vi "_CSMObj-Add Internal Registry Rule.vi"(8 "Error In":errorcluster caption="error in (no error)", 10 "Rule":string, 11 "CSMQ In":T1={"info"={"Module Name"="", "Requested Name"="", "Group Name"="", "Mode"=enum."Stand Alone", "Allowed Messages"=[]}, "Refs"={"WatchDogQ"=refnum, "CSMDataDVR"=refnum, "Queue"={"HPriorityQ"=refnum, "LowPriorityQ"=refnum}, "GroupDataDVR"=refnum, "TagMap"=refnum, "ExitEvent"=refnum, "NewStateEvent"=refnum, "StatusEvent"=refnum, "InterruptEvent"=refnum}}) -> (0 "error out":errorcluster, 3 "CSMQ Out":T1={"info"={"Module Name"="", "Requested Name"="", "Group Name"="", "Mode"=enum."Stand Alone", "Allowed Messages"=[]}, "Refs"={"WatchDogQ"=refnum, "CSMDataDVR"=refnum, "Queue"={"HPriorityQ"=refnum, "LowPriorityQ"=refnum}, "GroupDataDVR"=refnum, "TagMap"=refnum, "ExitEvent"=refnum, "NewStateEvent"=refnum, "StatusEvent"=refnum, "InterruptEvent"=refnum}})   [LabVIEW 2017, in "Communicable State Machine.lvlib"]
uses:
  Communicable State Machine.lvlib
  _CSMObj.ctl
  _CSMObj-Info.ctl
  Typedef/_CSM_MODE.ctl
  _CSMObj-Refs.ctl
  _CSMObj-Data.ctl
  Priority Queue/Priority Queue.ctl
  Typedef/_Cross CSM State Data.ctl
  Typedef/_CSM_MSG_TYPE.ctl
  Typedef/_Cross CSM State Response.ctl
  Typedef/_CSM_Response Source Message.ctl
  Priority Queue/def-Data(LowPRI-Q).ctl
  _CSMObj-ModeData.ctl
  Typedef/_CSM Status Change Event Data.ctl
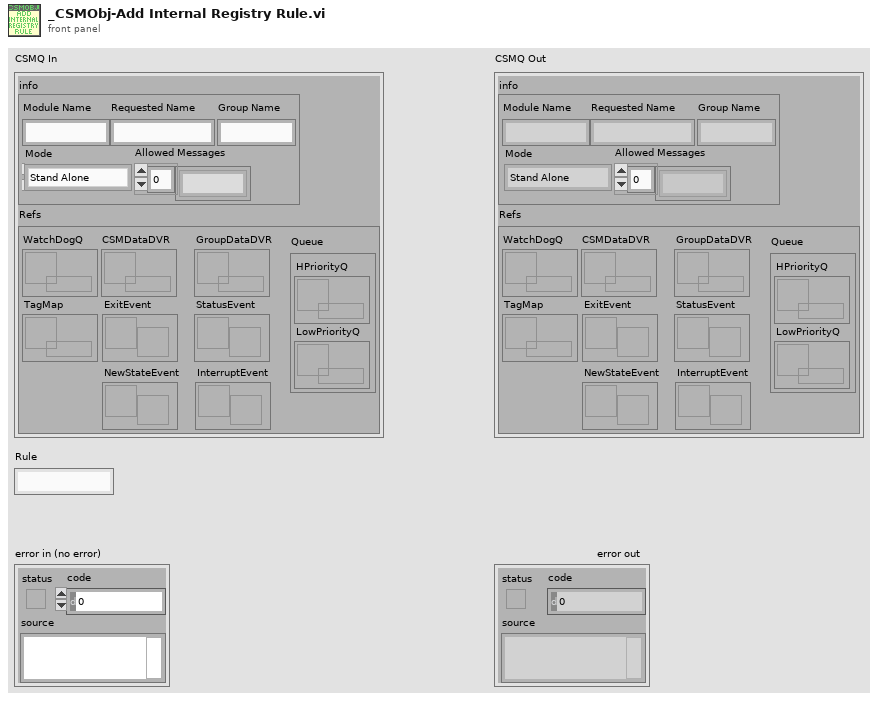
[diagram p1: front panel]
types:
  T1 = typedef "Communicable State Machine.lvlib/_CSMObj.ctl" = cluster{"info":T2, "Refs":T4}
  T2 = typedef "Communicable State Machine.lvlib/_CSMObj-Info.ctl" = cluster{"Module Name":string, "Requested Name":string, "Group Name":string, "Mode":T3, "Allowed Messages":string[]}
  T3 = typedef "Communicable State Machine.lvlib/_CSM_MODE.ctl" = enum16{"Not Exist", "Stand Alone", "CSM", "Worker", "Worker Agent", "Chain Node", "Chain"}
  T4 = typedef "Communicable State Machine.lvlib/_CSMObj-Refs.ctl" = cluster{"WatchDogQ":refnum<queue>, "CSMDataDVR":refnum<data-value>, "Queue":T5, "GroupDataDVR":refnum<data-value>, "TagMap":refnum<data-value>, "ExitEvent":refnum<user-event>, "NewStateEvent":refnum<user-event>, "StatusEvent":refnum<user-event>, "InterruptEvent":refnum<user-event>}
  T5 = typedef "Communicable State Machine.lvlib/Priority Queue.ctl" = cluster{"HPriorityQ":refnum<queue>, "LowPriorityQ":refnum<queue>}
  T6 = typedef "Communicable State Machine.lvlib/_CSMObj-Data.ctl" = cluster{"RemoteMessge?":bool, "error":errorcluster, "Return State":string, "Initialized":enum16{"Initializing", "Ready", "Exiting"}, "InternalRegistryRules":string[]}
  T7 = typedef "Communicable State Machine.lvlib/_CSMObj-ModeData.ctl" = cluster{"CSMDataDVR":refnum<data-value>[], "PriorityQueues":T5[], "Messages of Chain Nodes":cluster{"Module Name":string, "Allowed Messages":string[]}[], "Chain Message Mapping Map":variant, "SharedRegistryRules":string[]}
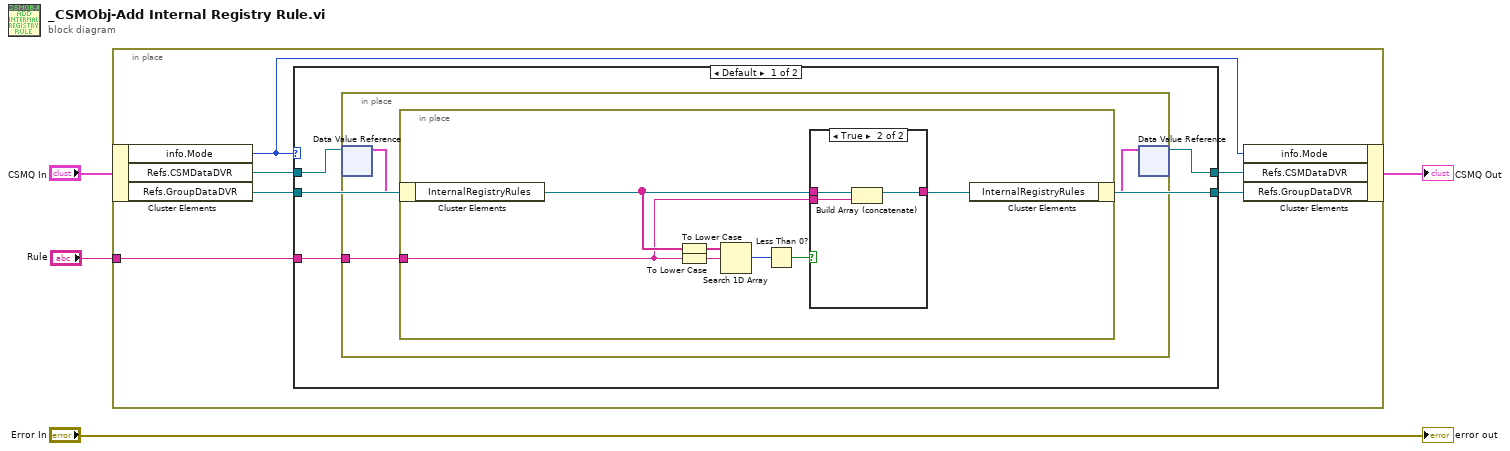
[diagram p0: block diagram]
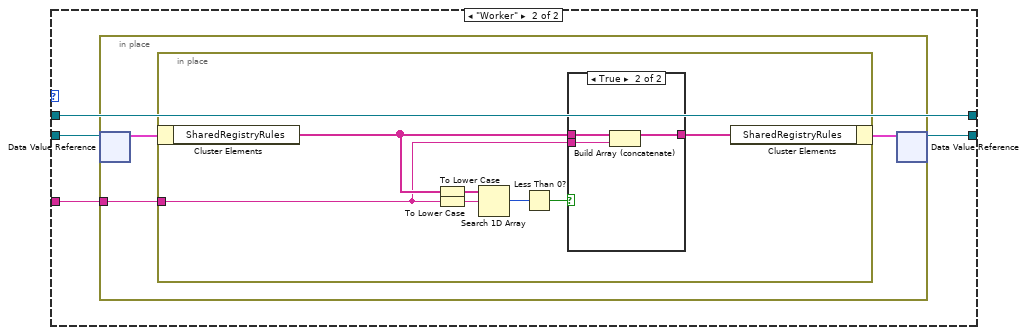
[diagram p3: hidden frame]
diagram:
  n1 = in-place "In Place Element Structure" {
    in-place-border: "Rule" -> [w8]
    n2 = in-place-cluster #1("CSMQ In") -> ("info.Mode"=w5:T3, "Refs.CSMDataDVR"=w7:refnum<data-value>, "Refs.GroupDataDVR"=w10:refnum<data-value>)
    n3 = case shown="Default" w5 {
      tunnel: w10 -> [w11 w30]
      tunnel: [w11 w29] -> w9
      tunnel: w8 -> [w14 w32]
      tunnel: w7 -> [w13 w31]
      tunnel: [w12 w31] -> w6
      frame Default {
        n4 = in-place {
          in-place-border: w14 -> [w17]
          n5 = in-place-dvr #2(w13) -> (w16:T6)  [unwired: 1 out]
          n6 = in-place {
            in-place-border: w17 -> [w20]
            n7 = in-place-cluster #3(w16) -> ("InternalRegistryRules"=w22:string[])
            n8 = To Lower Case(string=w22) -> (all lower case string=w24:string[])
            n9 = To Lower Case(string=w20) -> (all lower case string=w23:string)
            n10 = Search 1D Array(1D array=w24, element=w23) -> (index of element=w19:i32)  [unwired: 1 in]
            n11 = Less Than 0?(x=w19) -> (x < 0?=w18:bool)
            n12 = case shown="True" w18 {
              tunnel: w22 -> [w25 w28]
              tunnel: [w25 w27] -> w21
              tunnel: w20 -> [_ w26]
              frame False {
              }
              frame True {
                n13 = Build Array (concatenate)(w28, w26) -> (w27:string[])
              }
            }
            n14 = in-place-cluster #3("InternalRegistryRules"=w21) -> (w15:T6)
          }
          n15 = in-place-dvr #2(w15) -> (w12:refnum<data-value>)  [unwired: 1 out]
        }
      }
      frame "Worker" {
        n16 = in-place {
          in-place-border: w32 -> [w35]
          n17 = in-place-dvr #4(w30) -> (w34:T7)  [unwired: 1 out]
          n18 = in-place {
            in-place-border: w35 -> [w38]
            n19 = in-place-cluster #5(w34) -> ("SharedRegistryRules"=w40:string[])
            n20 = To Lower Case(string=w40) -> (all lower case string=w42:string[])
            n21 = To Lower Case(string=w38) -> (all lower case string=w41:string)
            n22 = Search 1D Array(1D array=w42, element=w41) -> (index of element=w37:i32)  [unwired: 1 in]
            n23 = Less Than 0?(x=w37) -> (x < 0?=w36:bool)
            n24 = case shown="True" w36 {
              tunnel: w40 -> [w43 w46]
              tunnel: [w43 w45] -> w39
              tunnel: w38 -> [_ w44]
              frame False {
              }
              frame True {
                n25 = Build Array (concatenate)(w46, w44) -> (w45:string[])
              }
            }
            n26 = in-place-cluster #5("SharedRegistryRules"=w39) -> (w33:T7)
          }
          n27 = in-place-dvr #4(w33) -> (w29:refnum<data-value>)  [unwired: 1 out]
        }
      }
    }
    n28 = in-place-cluster #1("info.Mode"=w5, "Refs.CSMDataDVR"=w6, "Refs.GroupDataDVR"=w9) -> (→"CSMQ Out":T1)
  }
  "error out" <- "Error In"
